vi "IR Limiter.vi"(0 "IR LO SET resistance value(M£[)":u16=2 min=1 max=9999, 5 "IR HI SET resistance value(M£[)":u16=9999 min=2 max=9999, 7 "IR Test Time(S)":sgl=1.0 min=1 max=999.9 format="%.1f", 9 "Ramp Time":sgl=0.1 min=0.1 max=999.9 format="%.1f", 11 "IR voltage(kV)":sgl=0.1 min=0.0499 max=1.0001 step=0.05 format="%.2f") -> (4 "IR voltage(kV)":string, 6 "IR Test Time(S)":string, 8 "IR LO SET":string, 10 "IR HI SET":string, 15 "Ramp Time":string)   [LabVIEW 2021]
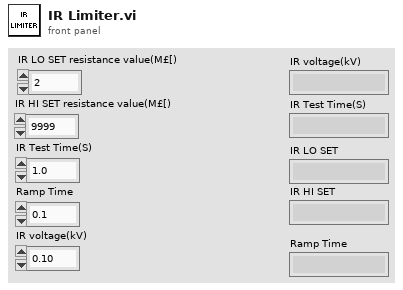
[diagram p1: front panel]
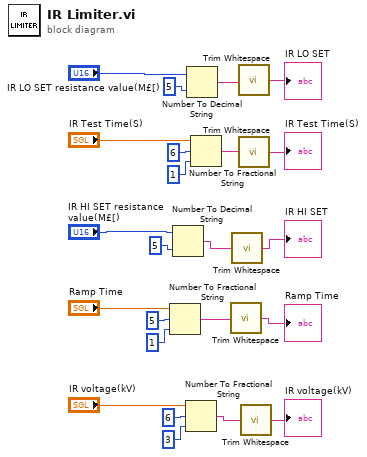
[diagram p0: block diagram]
diagram:
  n1 = Number To Fractional String(number="Ramp Time", width (-)=i16 5, precision (6)=i16 1) -> (F-format string=w3:string)  [unwired: 1 in]
  n2 = Number To Decimal String(number="IR HI SET resistance value(M£[)", width (-)=i16 5) -> (decimal integer string=w5:string)
  n3 = Number To Fractional String(number="IR voltage(kV)", width (-)=i16 6, precision (6)=i16 3) -> (F-format string=w8:string)  [unwired: 1 in]
  n4 = Number To Decimal String(number="IR LO SET resistance value(M£[)", width (-)=i16 5) -> (decimal integer string=w10:string)
  n5 = Number To Fractional String(number="IR Test Time(S)", width (-)=i16 6, precision (6)=i16 1 ("width (-)")) -> (F-format string=w9:string)  [unwired: 1 in]
  n6 = call <vilib>:"Trim Whitespace.vi"("string"=w3) -> ("trimmed string"=→"Ramp Time":string)  [unwired: 1 in]
  n7 = call <vilib>:"Trim Whitespace.vi"("string"=w5) -> ("trimmed string"=→"IR HI SET":string)  [unwired: 1 in]
  n8 = call <vilib>:"Trim Whitespace.vi"("string"=w10) -> ("trimmed string"=→"IR LO SET":string)  [unwired: 1 in]
  n9 = call <vilib>:"Trim Whitespace.vi"("string"=w9) -> ("trimmed string"=→"IR Test Time(S)":string)  [unwired: 1 in]
  n10 = call <vilib>:"Trim Whitespace.vi"("string"=w8) -> ("trimmed string"=→"IR voltage(kV)":string)  [unwired: 1 in]
